vi "Create MM Cluster.vi"(8 "error out":errorcluster, 11 "Channel Refs":T4[](array[typedef]) format="%.0x") -> (0 "error out 2":errorcluster, 3 "MM Data":T1)   [LabVIEW 2023, in "Vires VTD System Explorer.lvlib"]
uses:
  Vires VTD System Explorer.lvlib
  <vilib>/NI VeriStand/Custom Device API/Custom Device Item Ref.ctl
  MM/MM Data.ctl
  MM/MM Objects.ctl
  MM/MM Object.ctl
  <vilib>/NI VeriStand/Custom Device API/Get Item Property (Variant).vi
  <vilib>/NI VeriStand/Custom Device API/Custom Device API.lvlib
  MM/MM.lvlib
  Shared/Vires VTD Shared.lvlib
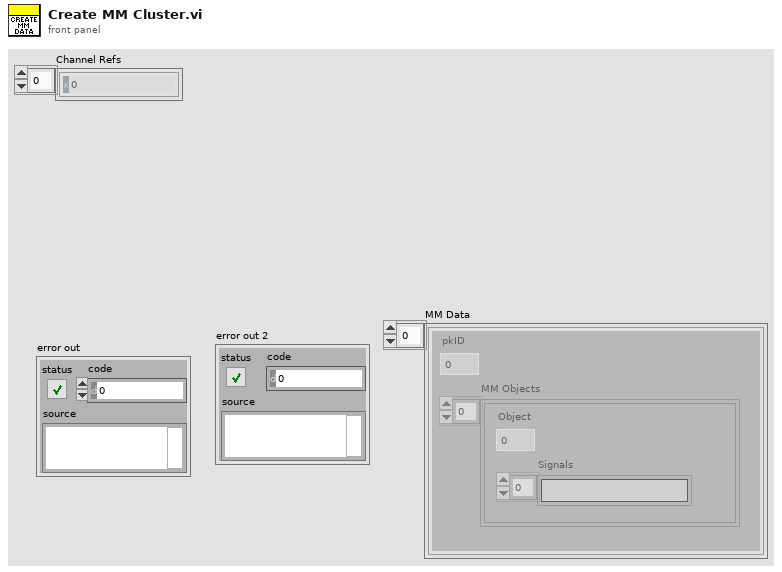
[diagram p1: front panel]
types:
  T1 = typedef "Vires VTD Shared.lvlib/MM Data.ctl" = T2[]
  T2 = typedef "MM.lvlib/MM Objects.ctl" = cluster{"pkID":i32, "MM Objects":T3[]}
  T3 = typedef "MM.lvlib/MM Object.ctl" = cluster{"Object":i32, "Signals":string[]}
  T4 = typedef "Custom Device API.lvlib/Custom Device Item Ref.ctl" = u64
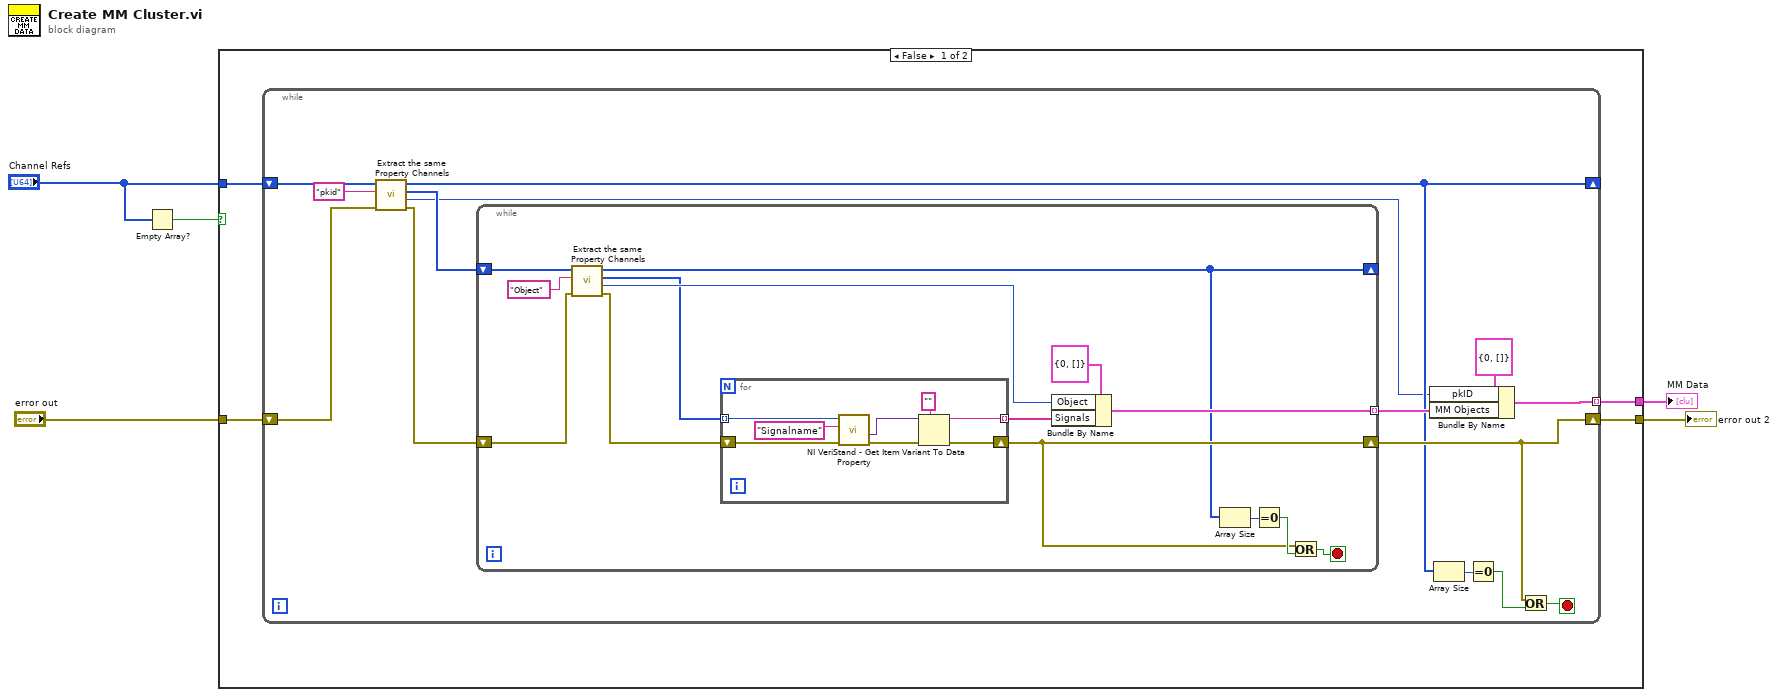
[diagram p0: block diagram]
diagram:
  n1 = Empty Array?(array="Channel Refs") -> (empty?=w2:bool)
  n2 = case shown="False" w2 {
    tunnel: "Channel Refs" -> [w9 _]
    tunnel: "error out" -> [w8 w46]
    tunnel: [w7 w46] -> w4
    tunnel: [w6 _] -> w1
    frame False {
      n3 = while {
        shift-right: [w14] -> _
        shift-left: w9 -> [w15]
        shift-right: [w20] -> w7
        shift-left: w8 -> [w12]
        tunnel: [w19] -> w6 mode=indexing
        stop <- w21 stop-if-true
        n4 = call "Extract the same Property Channels.vi"("error in (no error)"=w12, "Property Name"="pkid", "Channel Refs in"=w15) -> ("error out"=w11:errorcluster, "Property Value"=w10:u8, "Extracted the same pkid Channel Refs"=w13:T4[], "Channel Refs Remaining"=w14:T4[])  [unwired: 5 in]
        n5 = while {
          shift-right: [w27] -> _
          shift-left: w13 -> [w29]
          shift-right: [w33] -> w20
          shift-left: w11 -> [w28]
          tunnel: [w32] -> w17 mode=indexing
          stop <- w36 stop-if-true
          n6 = call "Extract the same Property Channels.vi"("error in (no error)"=w28, "Property Name"="Object", "Channel Refs in"=w29) -> ("error out"=w26:errorcluster, "Property Value"=w25:u8, "Extracted the same pkid Channel Refs"=w24:T4[], "Channel Refs Remaining"=w27:T4[])  [unwired: 5 in]
          n7 = for {
            tunnel: w24 -> [w43] mode=indexing
            shift-right: [w41] -> w33
            shift-left: w26 -> [w44]
            tunnel: [w38] -> w37 mode=indexing
            n8 = call-poly <vilib>:"NI VeriStand - Get Item Property.vi"("error in (no error)"=w44, "Property Name"="Signalname", "Item Ref in"=w43) -> ("error out"=w40:errorcluster, "Value"=w39:variant)  [unwired: 5 in, 2 out]
            n9 = Variant To Data(error in=w40, type="" ("Property Name"), Variant=w39) -> (data=w38:string, error out=w41:errorcluster)
          }
          n10 = Bundle By Name(cluster=T3 {"Object"=0, "Signals"=[]} ("RDB Player Object"), "Object"=w25, "Signals"=w37) -> (w32:T3)
          n11 = Array Size(array=w27) -> (size(s)=w35:i32)
          n12 = Equal To 0?(x=w35) -> (x = 0?=w34:bool)
          n13 = Or(x=w33, y=w34) -> (x .or. y?=w36:bool)
        }
        n14 = Bundle By Name(cluster=T2 {"pkID"=0, "MM Objects"=[]} ("MM Objects"), "pkID"=w10, "MM Objects"=w17) -> (w19:T2)
        n15 = Array Size(array=w14) -> (size(s)=w22:i32)
        n16 = Equal To 0?(x=w22) -> (x = 0?=w23:bool)
        n17 = Or(x=w20, y=w23) -> (x .or. y?=w21:bool)
      }
    }
    frame True {
    }
  }
  "error out 2" <- w4
  "MM Data" <- w1
